vi "Test_sqliteADONet_dist.vi"() -> ()   [LabVIEW 2026]
uses:
  <vilib>/Viviota/shared/ORM.lvlibp/TypeMap/TypeMap.lvclass
  <vilib>/Viviota/shared/ORM_lib.lvlibp/ObjectRow/ObjectLUT.lvclass
  <vilib>/numeric/Random Number (Range) I64.vi
  <vilib>/numeric/Random Number (Range) DBL.vi
  f3693442-7653-4e44-a421-498bef5f0c13.vi
  <vilib>/Analysis/baseanly.llb/Mean (DBL).vi
  <vilib>/numeric/sub_Random U32.vi
  <vilib>/Viviota/shared/ORM_ADONet.lvlibp/ADOMapper/ADOMapper.lvclass
  <vilib>/JDP Science/JSONtext/Variant to JSON Text.vi
  <vilib>/Viviota/shared/ORM_lib.lvlibp/ObjectRow/Write LUT.vi
  <vilib>/Viviota/shared/ORM_DBC_Sqlite_netCore.lvlibp/Sqlite Connect.vi
  <vilib>/Viviota/shared/ORM_sqlite_jdp.lvlibp/dbc/sqlite Connect.vi
  <vilib>/Viviota/shared/ORM_DBC_Sqlite.lvlibp/Sqlite Connect.vi
  <vilib>/Viviota/shared/ORM.lvlibp/SqlMapper/Read DbConnection.vi
  <vilib>/Viviota/shared/ORM.lvlibp/DbConnection/Write SupportTX.vi
  <vilib>/Viviota/shared/ORM.lvlibp/SqlMapper/Write DbConnection.vi
  <vilib>/Viviota/shared/ORM.lvlibp/TypeMap/Write Table Name.vi
  <vilib>/Viviota/shared/ORM.lvlibp/TypeMap/Write Autokey.vi
  <vilib>/Viviota/shared/ORM.lvlibp/TypeMap/Write ExcludeIDFromQueryParam.vi
  <vilib>/Viviota/shared/ORM_lib.lvlibp/ObjectRow/Read LUT.vi
  <vilib>/JDP Science/JSONtext/LVClass Serializer/JSONtext LVClass Serializer.lvclass
  <vilib>/Viviota/shared/ORM_ADONetCore.lvlibp/ADOMapper/ADOMapper.lvclass
  <vilib>/Viviota/shared/ORM.lvlibp/DbConnection/DbConnection.lvclass
  <vilib>/Viviota/shared/ORM.lvlibp/SqlMapper/SqlMapper.lvclass
  <vilib>/Analysis/NI_AALBase.lvlib
  <vilib>/Viviota/Viviota ORM - NetCore Connections/dotNetCore/NetCore_API/ORM_API_NetCore.lvlib
  <vilib>/Viviota/shared/ORM_DBC_Sqlite_netCore.lvlibp/DBC.lvclass
  <vilib>/Viviota/Viviota ORM - Direct Connections/DirectConnections/API/ORM_API_jdp.lvlib
  <vilib>/Viviota/shared/ORM_sqlite_jdp.lvlibp/dbc/DBC.lvclass
  <vilib>/Viviota/Viviota ORM/ORM_API/ORM_API.lvlib
  <vilib>/Viviota/shared/ORM_DBC_Sqlite.lvlibp/DBC.lvclass
panel:
  out "error out":errorcluster
  out "mean 3":dbl format="%0.6f"
  out "mean 2":dbl format="%0.6f"
  out "mean":dbl format="%0.6f"
  out "x-y":dbl[](array[numeric])
  out "Array 2":dbl[](array[numeric])
  out "Array":dbl[](array[numeric])
  out "LUT 2":variant[](array[variant])
  out "LUT":variant[](array[variant])
  out "id":i32[](array[numeric])
  # "0.019\n0.081\n0.034"
  # "0.013\n0.0072\n0.00029"
  # "0.01723\n0.0108\n0.0026"
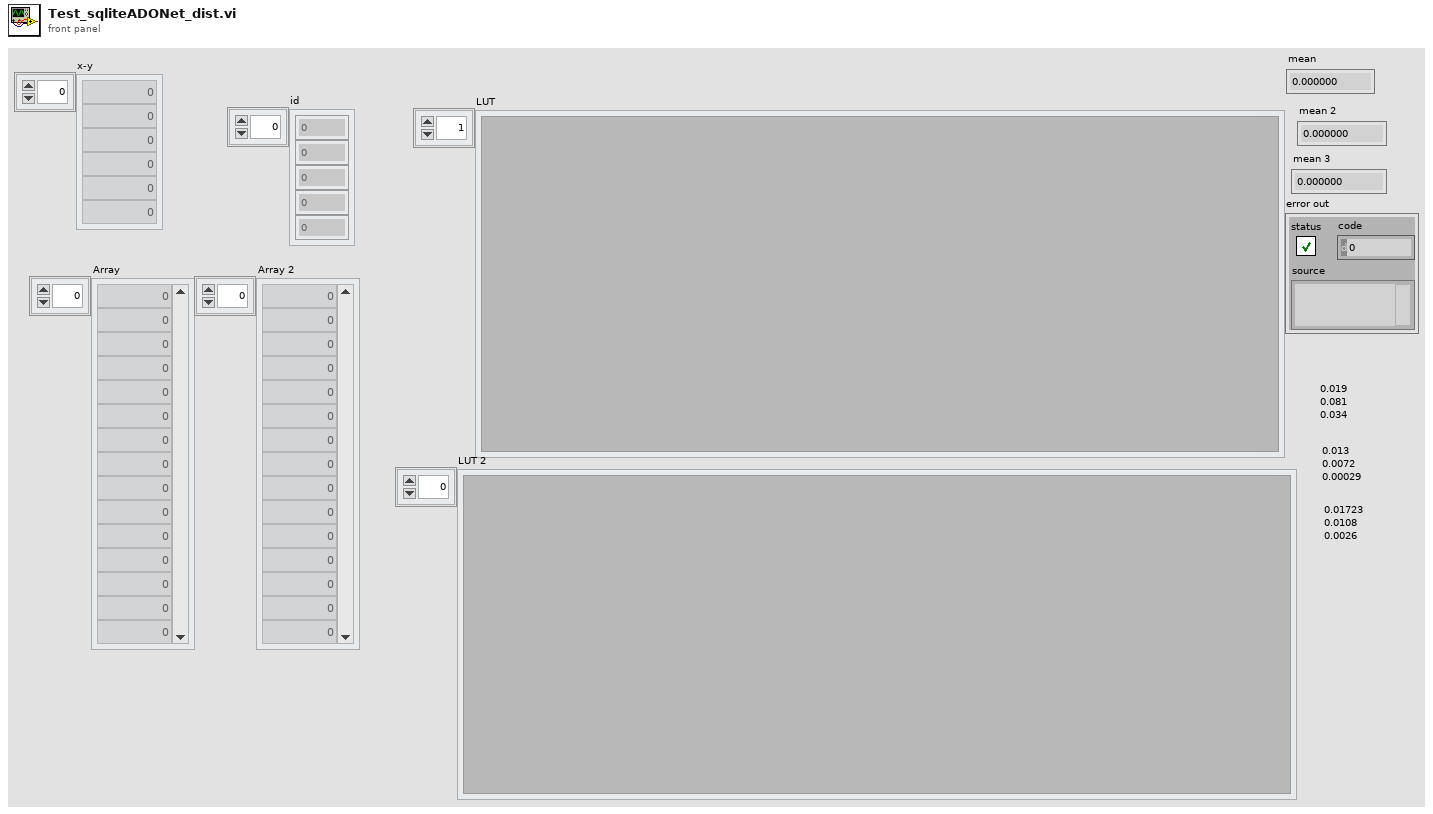
[diagram p1: front panel]
types:
  T1 = cluster{"Text":string, "Integer":i32, "dbl":dbl, "timestamp":timestamp}
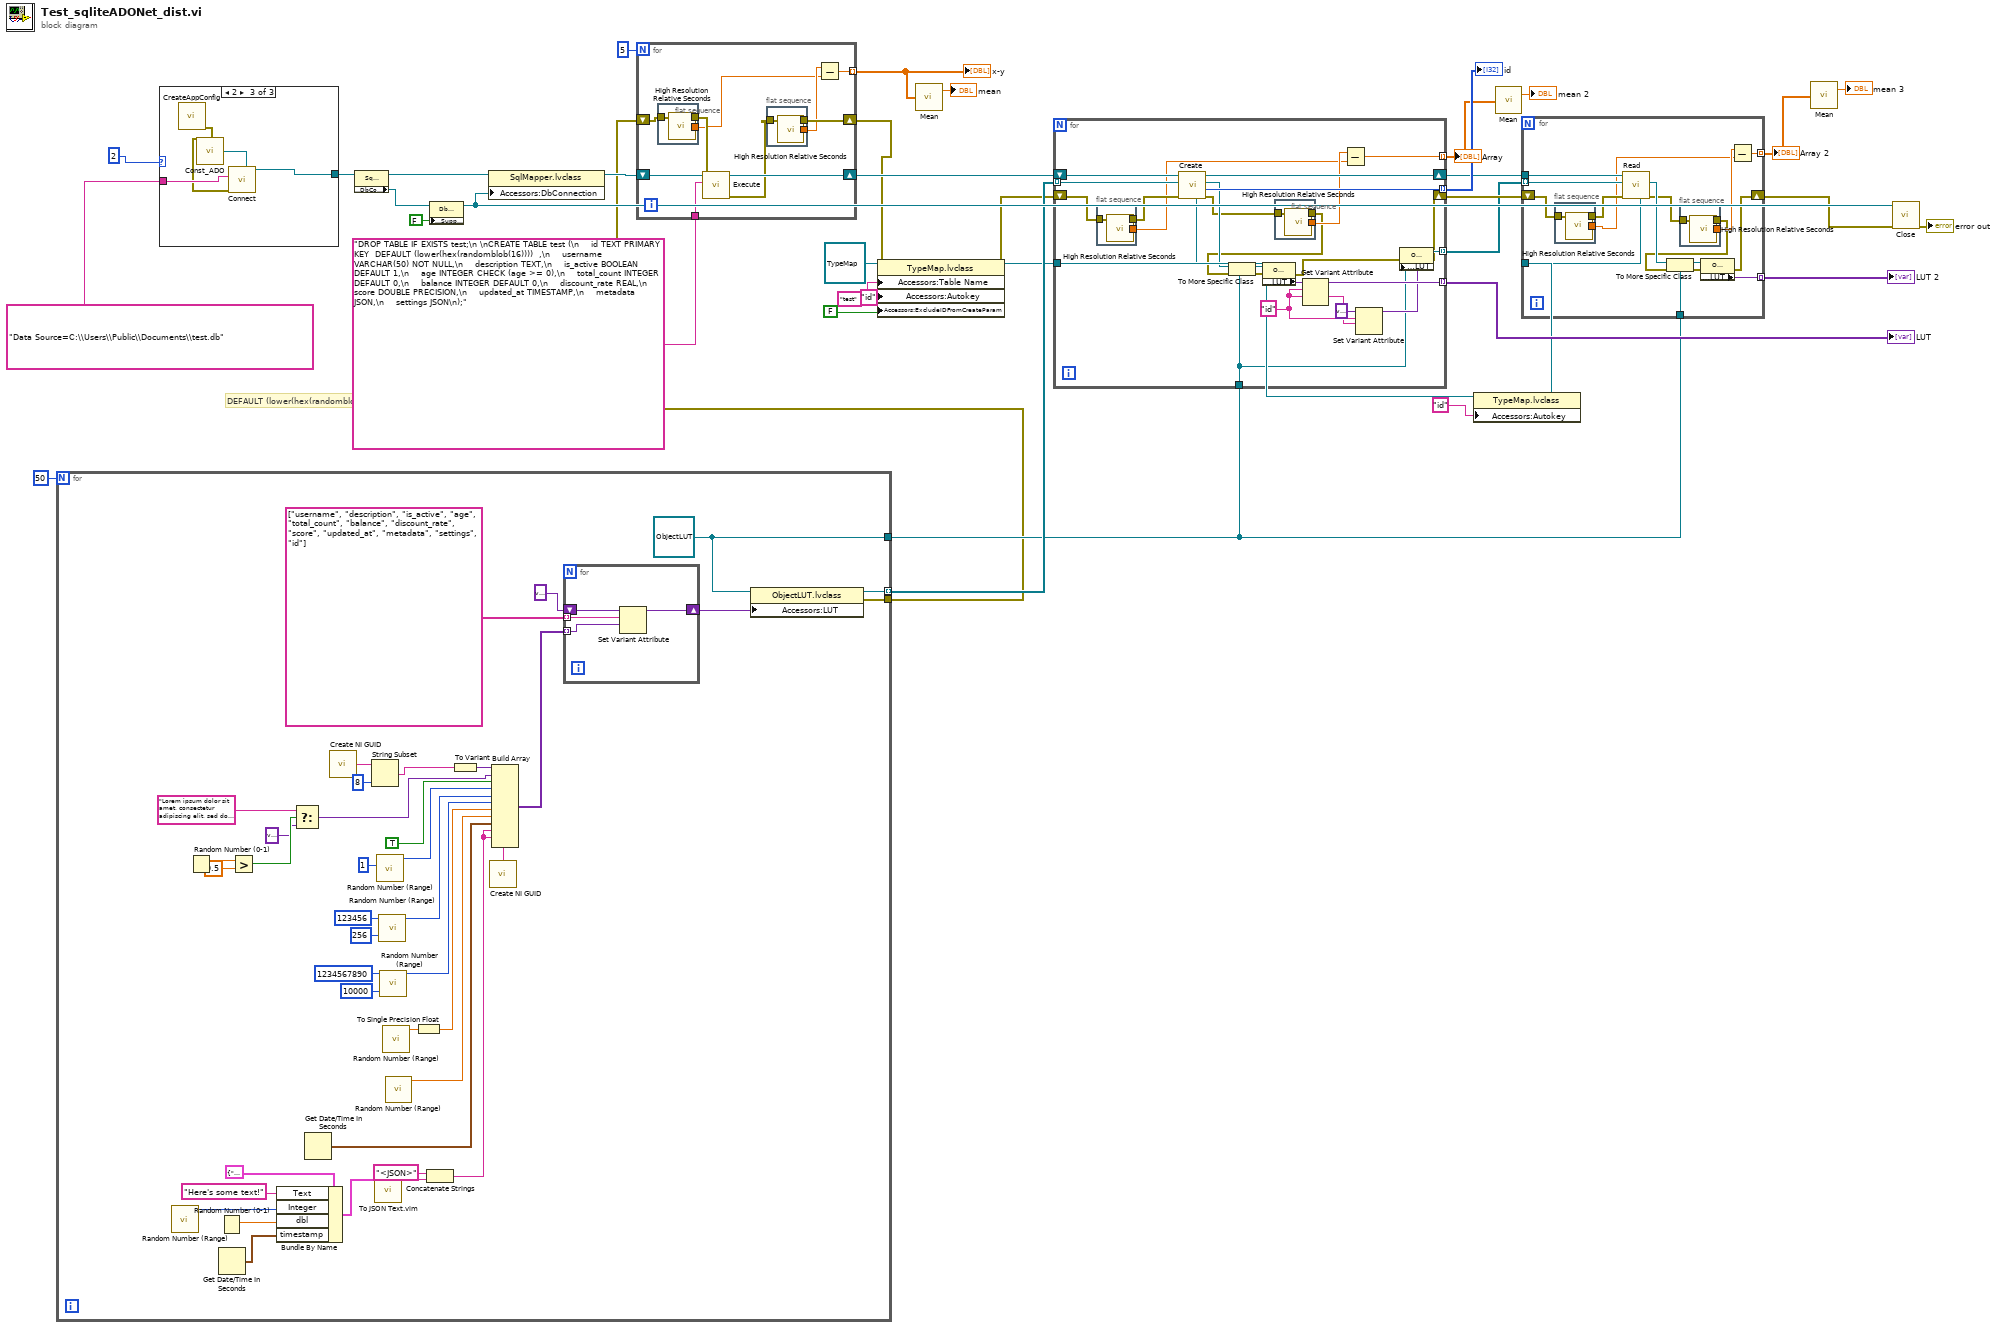
[diagram p0: block diagram]
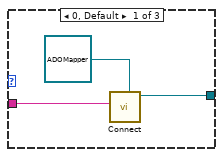
[diagram p2: hidden frame]
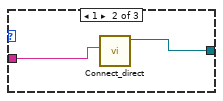
[diagram p3: hidden frame]
diagram:
  # "DEFAULT (lower(hex(randomblob(16))))"
  n1 = for {
    N: 50 -> [_]
    tunnel: [w48] -> w34 mode=indexing
    tunnel: [w47] -> w24
    tunnel: [w42] -> w20
    w47 = refnum<class "ObjectLUT.lvclass"> refnum ("ORM_lib.lvlibp:ObjectLUT.lvclass")
    n2 = call-poly <vilib>:"Random Number (Range).vi"() -> ("number"=w55:i64)  [unwired: 11 in]
    n3 = Random Number (0-1)() -> (number: 0 to 1=w63:dbl)
    n4 = Random Number (0-1)() -> (number: 0 to 1=w56:dbl)
    n5 = Get Date/Time In Seconds() -> (seconds since 1Jan1904=w57:timestamp)
    n6 = Greater?(x=w63, y=0.5) -> (0:w61:bool)
    n7 = Bundle By Name(cluster=T1 {"Text"="This is a test", "Integer"=0, "dbl"=0.0, "timestamp"=timestamp(0 s since 1904-01-01)}, "Text"="Here's some text!", "Integer"=w55, "dbl"=w56, "timestamp"=w57) -> (w53:T1)
    n8 = Select(t="Lorem ipsum dolor sit amet, consectetur adipiscing elit, sed do eiusmod tempor incididunt ut labore et dolore magna aliqua", s=w61, f=variant) -> (s? t:f=w39:variant)
    n9 = Get Date/Time In Seconds() -> (seconds since 1Jan1904=w54:timestamp)
    n10 = call <vilib>:"Create NI GUID.vi"() -> ("NI GUID"=w78:string)
    n11 = String Subset(string=w78, length (rest)=8 ("length (rest)")) -> (substring=w73:string)  [unwired: 1 in]
    n12 = call "To JSON Text.vim"("Anything"=w53) -> ("<JSON>"=w46:string)  [unwired: 9 in, 1 out]
    n13 = call-poly <vilib>:"Random Number (Range).vi"("lower bound (-100)"=i64 1) -> ("number"=w70:i64)  [unwired: 10 in]
    n14 = call-poly <vilib>:"Random Number (Range).vi"("lower bound (-100)"=i64 256, "upper bound (100)"=i64 123456) -> ("number"=w69:i64)  [unwired: 9 in]
    n15 = call-poly <vilib>:"Random Number (Range).vi"("lower bound (-100)"=i64 10000, "upper bound (100)"=i64 1234567890) -> ("number"=w68:i64)  [unwired: 9 in]
    n16 = call-poly <vilib>:"Random Number (Range).vi"() -> ("number"=w66:dbl)  [unwired: 11 in]
    n17 = call-poly <vilib>:"Random Number (Range).vi"() -> ("number"=w64:dbl)  [unwired: 11 in]
    n18 = To Single Precision Float(number=w66) -> (single precision float=w65:sgl)
    n19 = Concatenate Strings("<JSON>" ("string"), w46) -> (w45:string)
    n20 = To Variant(anything=w73) -> (Variant=w72:variant)
    n21 = call <vilib>:"Create NI GUID.vi"() -> ("NI GUID"=w40:string)
    n22 = Build Array(w72, w39, TRUE, w70, w69, w68, w65, w64, w54, w45, w45, w40) -> (w51:variant[])
    n23 = for {
      tunnel: string[] ["username", "description", "is_active", "age", "total_count", "balance", "discount_rate", "score", "updated_at", "metadata", "settings", "id"] -> [w82] mode=indexing
      tunnel: w51 -> [w81] mode=indexing
      shift-right: [w80] -> w49
      shift-left: variant -> [w79]
      n24 = Set Variant Attribute(Variant=w79, name=w82, value=w81) -> (Variant out=w80:variant)  [unwired: 1 in, 2 out]
    }
    n25 = property class="ObjectLUT.lvclass"(reference=w47, "Accessors:LUT"=w49) -> (reference out=w48:refnum<class "ObjectLUT.lvclass">, error out=w42:errorcluster)  [unwired: 1 in]
  }
  n26 = case shown="2" 2 {
    tunnel: "Data Source=C:\\Users\\Public\\Documents\\test.db" ("Connection String") -> [w85 w86 w89]
    tunnel: [w83 w87 w91] -> w4
    frame 0, Default {
      n27 = call-poly <vilib>:"Connect.vi"("SqlMapper Type"=refnum<class "ADOMapper.lvclass"> refnum ("ORM_ADONetCore.lvlibp:ADOMapper.lvclass"), "Connection String"=w85) -> ("SqlMapper out"=w83:refnum<class "ADOMapper.lvclass">)  [unwired: 8 in, 1 out]
    }
    frame 1 {
      n28 = call-poly <vilib>:"Connect_direct.vi"("Connection String"=w86) -> ("SqlMapper out"=w87:refnum<class "SqlMapper.lvclass">)  [unwired: 9 in, 1 out]
    }
    frame 2 {
      n29 = call <vilib>:"CreateAppConfig.vi"() -> ("error out"=w88:errorcluster)  [unwired: 11 in]
      n30 = call <vilib>:"Const_ADO.vi"() -> ("ADOMapper"=w90:refnum<class "ADOMapper.lvclass">)
      n31 = call-poly <vilib>:"Connect.vi"("SqlMapper Type"=w90, "error in (no error)"=w88, "Connection String"=w89) -> ("SqlMapper out"=w91:refnum<class "ADOMapper.lvclass">)  [unwired: 7 in, 1 out]
    }
  }
  n32 = property class="SqlMapper.lvclass"(reference=w4) -> (reference out=w2:refnum<class "SqlMapper.lvclass">, "Accessors:DbConnection"=w3:refnum<class "DbConnection.lvclass">)  [unwired: 1 in, 1 out]
  n33 = property class="DbConnection.lvclass"(reference=w3, "Accessors:SupportTX"=FALSE ("SupportTX")) -> (reference out=w35:refnum<class "DbConnection.lvclass">)  [unwired: 1 in, 1 out]
  n34 = property class="SqlMapper.lvclass"(reference=w2, "Accessors:DbConnection"=w35) -> (reference out=w37:refnum<class "SqlMapper.lvclass">)  [unwired: 1 in, 1 out]
  n35 = for {
    N: 5 -> [_]
    tunnel: "DROP TABLE IF EXISTS test;\n \nCREATE TABLE test (\n    id TEXT PRIMARY KEY  DEFAULT (lower(hex(randomblob(16))))  ,\n    username VARCHAR(50) NOT NULL,\n    description TEXT,\n    is_active BOOLEAN DEFAULT 1,\n    age INTEGER CHECK (age >= 0),\n    total_count INTEGER DEFAULT 0,\n    balance INTEGER DEFAULT 0,\n    discount_rate REAL,\n    score DOUBLE PRECISION,\n    updated_at TIMESTAMP,\n    metadata JSON,\n    settings JSON\n);" ("sql") -> [w100]
    tunnel: [w92] -> w17 mode=indexing
    shift-right: [w99] -> w26
    shift-left: w37 -> [w101]
    shift-right: [w95] -> w19
    shift-left: w20 -> [w98]
    n36 = flat-sequence {
      tunnel: [w105] -> w93
      tunnel: w98 -> [w104]
      tunnel: [w104] -> w97
      frame #0 {
        n37 = call <vilib>:"High Resolution Relative Seconds.vi"() -> ("relative seconds"=w105:dbl)
      }
    }
    n38 = call-dynamic "Execute.vi"("error in (no error)"=w97, "sql"=w100, "SqlMapper in"=w101) -> ("error out"=w96:errorcluster, "SqlMapper out"=w99:refnum<class "SqlMapper.lvclass">)  [unwired: 6 in, 1 out]
    n39 = flat-sequence {
      tunnel: [w103] -> w94
      tunnel: w96 -> [w102]
      tunnel: [w102] -> w95
      frame #0 {
        n40 = call <vilib>:"High Resolution Relative Seconds.vi"() -> ("relative seconds"=w103:dbl)
      }
    }
    n41 = Subtract(x=w94, y=w93) -> (x-y=w92:dbl)
  }
  "x-y" <- w17
  n42 = property class="TypeMap.lvclass"(reference=refnum<class "TypeMap.lvclass"> refnum ("TypeMap in"), error in=w19, "Accessors:Table Name"="test" ("Table Name"), "Accessors:Autokey"="id" ("Autokey"), "Accessors:ExcludeIDFromCreateParam"=FALSE ("ExcludeIDFromCreateParam")) -> (reference out=w25:refnum<class "TypeMap.lvclass">, error out=w11:errorcluster)
  n43 = call-poly <vilib>:"Mean.vi"("X"=w17) -> ("mean"=→"mean":dbl)  [unwired: 1 out]
  n44 = for {
    tunnel: w34 -> [w129] mode=indexing
    tunnel: w25 -> [w128]
    tunnel: [w127] -> w31 mode=indexing
    tunnel: w24 -> [w117]
    tunnel: [w122] -> w30 mode=indexing
    shift-right: [w106] -> w28
    shift-left: w11 -> [w115]
    tunnel: [w116] -> w27 mode=indexing
    shift-right: [w112] -> w21
    shift-left: w26 -> [w130]
    tunnel: [w109] -> w13 mode=indexing
    w120 = "id" ("name")
    n45 = flat-sequence {
      tunnel: [w134] -> w110
      tunnel: w115 -> [w133]
      tunnel: [w133] -> w114
      frame #0 {
        n46 = call <vilib>:"High Resolution Relative Seconds.vi"() -> ("relative seconds"=w134:dbl)
      }
    }
    n47 = call-dynamic "Create.vi"("TypeMap in"=w128, "error in (no error)"=w114, "object in"=w129, "SqlMapper in"=w130) -> ("error out"=w113:errorcluster, "id"=w127:i32, "object out"=w126:refnum<class>, "SqlMapper out"=w112:refnum<class "SqlMapper.lvclass">)  [unwired: 4 in]
    n48 = To More Specific Class(target class=w117, reference=w126, error in=w108) -> (specific class reference=w124:refnum<class "ObjectLUT.lvclass">, error out=w125:errorcluster)
    n49 = property class="ObjectLUT.lvclass"(reference=w124, error in=w125) -> (error out=w107:errorcluster, "Accessors:LUT"=w123:variant)  [unwired: 1 out]
    n50 = flat-sequence {
      tunnel: [w132] -> w111
      tunnel: w113 -> [w131]
      tunnel: [w131] -> w108
      frame #0 {
        n51 = call <vilib>:"High Resolution Relative Seconds.vi"() -> ("relative seconds"=w132:dbl)
      }
    }
    n52 = Get Variant Attribute(Variant=w123, name=w120, default value (empty Variant)=w120) -> (duplicate Variant=w122:variant, value=w119:string)  [unwired: 1 in, 2 out]
    n53 = Subtract(x=w111, y=w110) -> (x-y=w109:dbl)
    n54 = Set Variant Attribute(Variant=variant ("variant"), name=w120, value=w119) -> (Variant out=w118:variant)  [unwired: 1 in, 2 out]
    n55 = property class="ObjectLUT.lvclass"(reference=w117, error in=w107, "Accessors:LUT"=w118) -> (reference out=w116:refnum<class "ObjectLUT.lvclass">, error out=w106:errorcluster)
  }
  "id" <- w31
  "LUT" <- w30
  "Array" <- w13
  n56 = property class="TypeMap.lvclass"(reference=w25, "Accessors:Autokey"="id" ("Autokey")) -> (reference out=w9:refnum<class "TypeMap.lvclass">)  [unwired: 1 in, 1 out]
  n57 = call-poly <vilib>:"Mean.vi"("X"=w13) -> ("mean"=→"mean 2":dbl)  [unwired: 1 out]
  n58 = for {
    tunnel: w27 -> [w150] mode=indexing
    tunnel: w21 -> [w149]
    tunnel: w9 -> [w148]
    tunnel: w24 -> [w144]
    tunnel: [w143] -> w23 mode=indexing
    shift-right: [w135] -> w22
    shift-left: w28 -> [w142]
    tunnel: [w137] -> w12 mode=indexing
    n59 = flat-sequence {
      tunnel: [w154] -> w138
      tunnel: w142 -> [w153]
      tunnel: [w153] -> w141
      frame #0 {
        n60 = call <vilib>:"High Resolution Relative Seconds.vi"() -> ("relative seconds"=w154:dbl)
      }
    }
    n61 = call-dynamic "Read.vi"("TypeMap in"=w148, "error in (no error)"=w141, "object in"=w150, "SqlMapper in"=w149) -> ("error out"=w140:errorcluster, "Value"=w145:refnum<class>)  [unwired: 4 in, 2 out]
    n62 = To More Specific Class(target class=w144, reference=w145, error in=w136) -> (specific class reference=w147:refnum<class "ObjectLUT.lvclass">, error out=w146:errorcluster)
    n63 = flat-sequence {
      tunnel: [w152] -> w139
      tunnel: w140 -> [w151]
      tunnel: [w151] -> w136
      frame #0 {
        n64 = call <vilib>:"High Resolution Relative Seconds.vi"() -> ("relative seconds"=w152:dbl)
      }
    }
    n65 = property class="ObjectLUT.lvclass"(reference=w147, error in=w146) -> (error out=w135:errorcluster, "Accessors:LUT"=w143:variant)  [unwired: 1 out]
    n66 = Subtract(x=w139, y=w138) -> (x-y=w137:dbl)
  }
  "LUT 2" <- w23
  "Array 2" <- w12
  n67 = call-poly <vilib>:"Mean.vi"("X"=w12) -> ("mean"=→"mean 3":dbl)  [unwired: 1 out]
  n68 = call-dynamic "Close.vi"("error in (no error)"=w22, "DbConnection in"=w35) -> ("error out"=→"error out":errorcluster)  [unwired: 9 in]
